vi "Lire config compteurs.vi"(2 "error in":errorcluster, 3 "refnum":T1) -> (0 "error out":errorcluster, 1 "refnum out":T1)   [LabVIEW 2022 SP3]
uses:
  <vilib>/Utility/config.llb/Config Data RefNum.ctl
  <vilib>/Utility/config.llb/Read Key (String).vi
  Variables globales/Variable globale compteurs.vi
  <vilib>/Utility/config.llb/Read Key (Boolean).vi
  <vilib>/Utility/config.llb/Read Key (Double).vi
  <vilib>/Utility/config.llb/Read Key (I32).vi
  <vilib>/Utility/config.llb/NI_LVConfig.lvlib
panel:
  # "lecture fichier config compteurs"
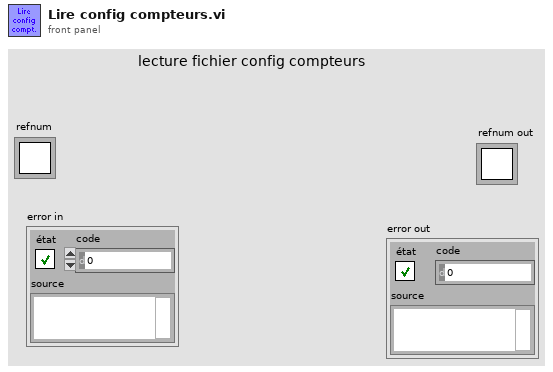
[diagram p1: front panel]
types:
  T1 = typedef "NI_LVConfig.lvlib/Config Data RefNum.ctl" = refnum<k1>
  T2 = cluster{"Nom tache compteurs":refnum<k21>, "Noms des compteurs":string[], "Sélection":bool[], "Init compteurs":dbl[], "Noms compteurs sélectionnés":string[]}
  T3 = cluster{"Nom tache compteurs":refnum<k21>, "Noms des compteurs":string[], "Selection":bool[], "Init compteurs":dbl[], "Noms compteurs selectionnes":string[]}
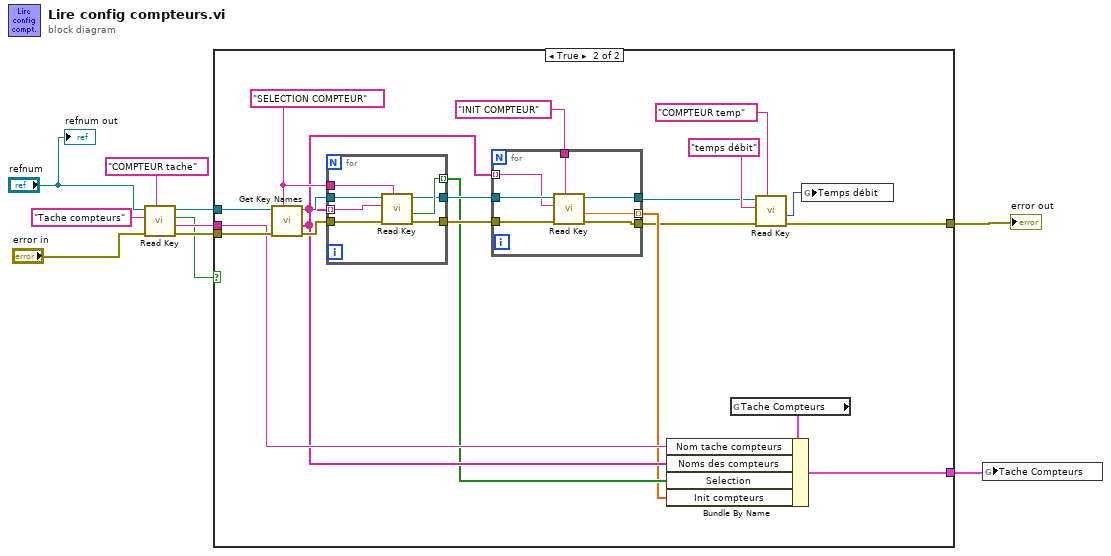
[diagram p0: block diagram]
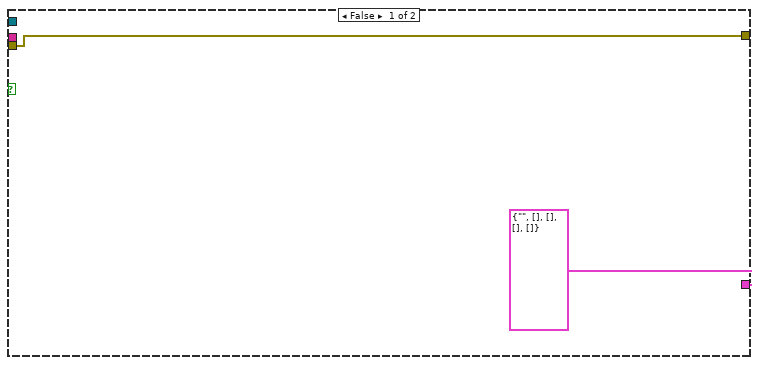
[diagram p2: hidden frame]
diagram:
  n1 = call-poly <vilib>:"Read Key.vi"("section"="COMPTEUR tache", "error in (no error)"="error in", "key"="Tache compteurs", "refnum"="refnum") -> ("error out"=w7:errorcluster, "value"=w5:string, "found?"=w1:bool, "refnum out"=w8:T1)  [unwired: 4 in]
  n2 = case shown="True" w1 {
    tunnel: [w12 w16] -> w10
    tunnel: w8 -> [_ w26]
    tunnel: w7 -> [w12 w25]
    tunnel: w5 -> [_ w23]
    tunnel: [T2 {"Nom tache compteurs"="", "Noms des compteurs"=[], "Sélection"=[], "Init compteurs"=[], "Noms compteurs sélectionnés"=[]} ("Tache Compteurs") w19] -> w4
    frame False {
    }
    frame True {
      w32 = "SELECTION COMPTEUR" ("section")
      n3 = call <vilib>:"Get Key Names.vi"("section"=w32, "error in (no error)"=w25, "refnum"=w26) -> ("error out"=w30:errorcluster, "key names"=w22:string[], "refnum out"=w31:T1)  [unwired: 5 in, 1 out]
      n4 = for {
        tunnel: w32 -> [w46]
        tunnel: w31 -> [w45]
        tunnel: w22 -> [w44] mode=indexing
        tunnel: w30 -> [w43]
        tunnel: [w42] -> w21 mode=indexing
        tunnel: [w41] -> w27
        tunnel: [w40] -> w28
        n5 = call-poly <vilib>:"Read Key.vi"("section"=w46, "error in (no error)"=w43, "key"=w44, "refnum"=w45) -> ("error out"=w40:errorcluster, "value"=w42:bool, "refnum out"=w41:T1)  [unwired: 4 in, 1 out]
      }
      n6 = for {
        tunnel: w28 -> [w38]
        tunnel: "INIT COMPTEUR" ("section") -> [w36]
        tunnel: w27 -> [w39]
        tunnel: [w37] -> w14
        tunnel: w22 -> [w35] mode=indexing
        tunnel: [w34] -> w20 mode=indexing
        tunnel: [w33] -> w13
        n7 = call-poly <vilib>:"Read Key.vi"("section"=w36, "error in (no error)"=w38, "key"=w35, "refnum"=w39) -> ("error out"=w33:errorcluster, "value"=w34:dbl, "refnum out"=w37:T1)  [unwired: 4 in, 1 out]
      }
      n8 = global read "Variable globale compteurs.vi" "Tache Compteurs"() -> (w24:T3)
      n9 = Bundle By Name(cluster=w24, "Nom tache compteurs"=w23, "Noms des compteurs"=w22, "Selection"=w21, "Init compteurs"=w20) -> (w19:T3)
      n10 = call-poly <vilib>:"Read Key.vi"("section"="COMPTEUR temp", "error in (no error)"=w13, "key"="temps débit", "refnum"=w14) -> ("error out"=w16:errorcluster, "value"=w15:i32)  [unwired: 4 in, 2 out]
      n11 = global write "Variable globale compteurs.vi" "Temps débit"(w15) -> ()
    }
  }
  "error out" <- w10
  n12 = global write "Variable globale compteurs.vi" "Tache Compteurs"(w4) -> ()
  "refnum out" <- "refnum"
